vi "Update Icon Textvi.vi"(9 "Icon Color":u32(colorbox)=13631442, 10 "Suubsystem Name":string="Drive", 11 "vi reference":refnum<vi>) -> (3 "VI Refnum out":refnum<vi>)   [LabVIEW 2023]
uses:
  <vilib>/LabVIEW Icon API/lv_icon/Controls/Graphic.ctl
  <vilib>/LabVIEW Icon API/lv_icon/Classes/Layer/Layer.lvclass
  <vilib>/LabVIEW Icon API/lv_icon/Controls/Layer.ctl
  <vilib>/LabVIEW Icon API/lv_icon/Classes/Icon/Icon.lvclass
  <vilib>/LabVIEW Icon API/lv_icon/Classes/Icon Framework/Icon Framework.lvclass
  <vilib>/LabVIEW Icon API/LabVIEW Icon API.lvlib
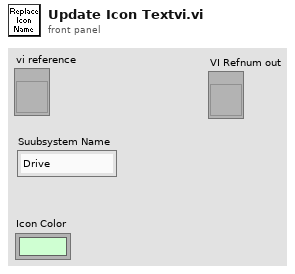
[diagram p1: front panel]
types:
  T1 = typedef "Layer.ctl" = cluster{"LayerIcon":picture, "LayerName":string, "Opacity":u8, "Visibility?":bool}
  T2 = cluster{"left":i16, "top":i16, "right":i16, "bottom":i16}
  T3 = typedef "Graphic.ctl" = cluster{"Rectangle":cluster{"left":i16, "top":i16, "right":i16, "bottom":i16}, "Path":path, "Image":picture, "Filter":string, "FileName":string}
  T4 = typedef "BodyText.ctl" = cluster{"Line 1 text":string, "Line 2 text":string, "Line 3 text":string, "Line 4 text":string, "Line 1 color":u32, "Line 2 color":u32, "Line 3 color":u32, "Line 4 color":u32, "Body Text Spec":cluster{"Font":T5, "Alignment":T6, "Size":u8}, "Center text vertically":bool, "Capitalize Text":bool}
  T5 = typedef "Font.ctl" = string
  T6 = typedef "Alignment.ctl" = u16
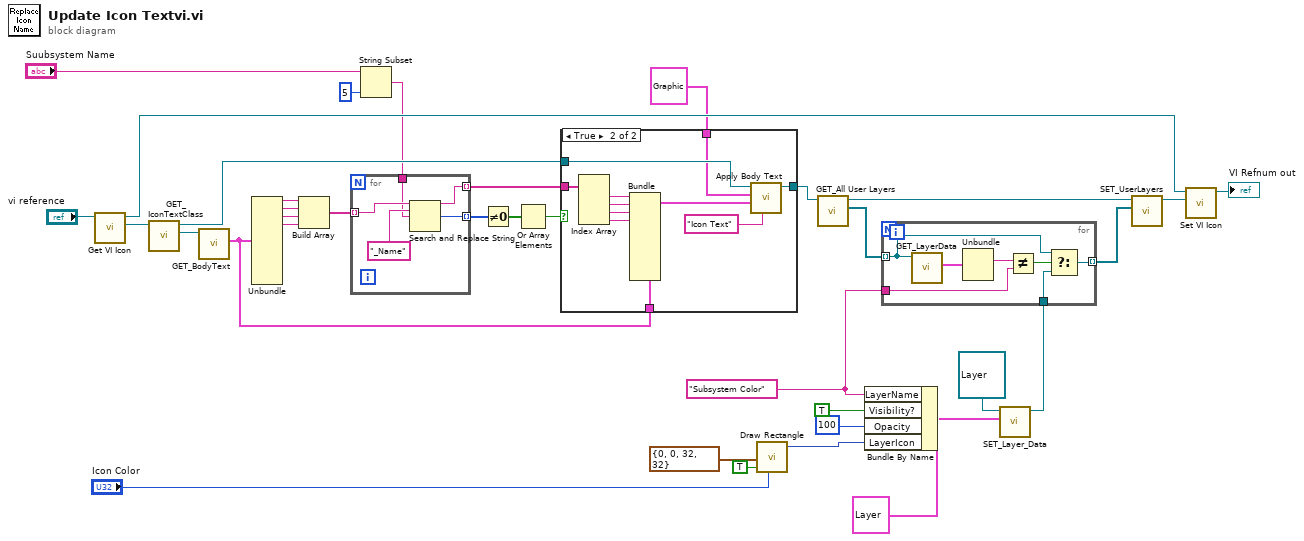
[diagram p0: block diagram]
diagram:
  w3 = "Subsystem Color" ("Layer name")
  n1 = call <vilib>:"Get VI Icon.vi"("VI Refnum in"="vi reference") -> ("Icon"=w36:refnum<class "Icon.lvclass">, "VI Refnum out"=w24:refnum<vi>)  [unwired: 8 in, 1 out]
  n2 = call-dynamic "GET_IconTextClass.vi"("Icon.lvclass in"=w36) -> ("Icon Framework.lvclass"=w35:refnum<class "Icon Framework.lvclass">, "Icon.lvclass out"=w25:refnum<class "Icon.lvclass">)  [unwired: 8 in, 1 out]
  n3 = call-dynamic "GET_BodyText.vi"("Icon Framework.lvclass in"=w35) -> ("Body Text"=w26:T4)  [unwired: 7 in, 3 out]
  n4 = Unbundle(w26) -> ("Line 1 text"=w31:string, "Line 2 text"=w32:string, "Line 3 text"=w33:string, "Line 4 text"=w34:string)  [unwired: 7 out]
  n5 = Build Array(w31, w32, w33, w34) -> (w30:string[])
  n6 = String Subset(string="Suubsystem Name", length (rest)=5 ("length (rest)")) -> (substring=w19:string)  [unwired: 1 in]
  n7 = for {
    tunnel: w30 -> [w40] mode=indexing
    tunnel: w19 -> [w39]
    tunnel: [w38] -> w29 mode=indexing
    tunnel: [w37] -> w27 mode=indexing
    n8 = Search and Replace String(input string=w40, search string="_Name", replace string=w39) -> (result string=w37:string, number of replacements=w38:i32)  [unwired: 5 in, 2 out]
  }
  n9 = Not Equal To 0?(x=w29) -> (x != 0?=w28:bool[])
  n10 = Or Array Elements(Boolean array=w28) -> (logical OR=w5:bool)
  n11 = case shown="True" w5 {
    tunnel: w27 -> [_ w53]
    tunnel: w26 -> [_ w52]
    tunnel: w25 -> [w42 w51]
    tunnel: T3 {"Rectangle"={"left"=0, "top"=0, "right"=0, "bottom"=0}, "Path"=path "", "Image"=bytes[0], "Filter"="", "FileName"=""} ("Path & Icon") -> [_ w50]
    tunnel: [w42 w43] -> w7
    frame False {
    }
    frame True {
      n12 = Index Array(array=w53) -> (element #1=w49:string, element #2=w48:string, element #3=w47:string, element #4=w46:string)  [unwired: 4 in]
      n13 = Bundle(cluster=w52, "Line 1 text"=w49, "Line 2 text"=w48, "Line 3 text"=w47, "Line 4 text"=w46) -> (w45:T4)  [unwired: 7 in]
      n14 = call <vilib>:"Apply Body Text.vi"("Layer name"="Icon Text", "Body test"=w45, "Path & Icon"=w50, "Icon in"=w51) -> ("Icon out"=w43:refnum<class "Icon.lvclass">)  [unwired: 5 in, 2 out]
    }
  }
  n15 = call <vilib>:"Draw Rectangle.vi"("rect"=T2 {"left"=0, "top"=0, "right"=32, "bottom"=32}, "fill?(F)"=TRUE, "color(black)"="Icon Color") -> ("new picture"=w11:picture)  [unwired: 6 in]
  n16 = call-dynamic "GET_All User Layers.vi"("Icon.lvclass in"=w7) -> ("User Layer"=w4:refnum<class "Layer.lvclass">[], "Icon.lvclass out"=w8:refnum<class "Icon.lvclass">)  [unwired: 8 in, 1 out]
  n17 = Bundle By Name(cluster=T1 {"LayerIcon"=bytes[0], "LayerName"="", "Opacity"=0, "Visibility?"=FALSE} ("Data"), "LayerName"=w3, "Visibility?"=TRUE, "Opacity"=u8 100, "LayerIcon"=w11) -> (w9:T1)
  n18 = call-dynamic "SET_Layer_Data.vi"("Data"=w9, "Layer.lvclass in"=refnum<class "Layer.lvclass"> refnum) -> ("Layer.lvclass out"=w2:refnum<class "Layer.lvclass">)  [unwired: 2 in, 7 out]
  n19 = for {
    tunnel: w4 -> [w56] mode=indexing
    tunnel: w3 -> [w59]
    tunnel: w2 -> [w55]
    tunnel: [w54] -> w1 mode=indexing
    n20 = call-dynamic "GET_LayerData.vi"("Layer.lvclass in"=w56) -> ("Data"=w60:T1)  [unwired: 6 in, 4 out]
    n21 = Unbundle(w60) -> ("LayerName"=w58:string)  [unwired: 3 out]
    n22 = Not Equal?(x=w58, y=w59) -> (x != y?=w57:bool)
    n23 = Select(t=w56, s=w57, f=w55) -> (s? t:f=w54:refnum<class "Layer.lvclass">)
  }
  n24 = call-dynamic "SET_UserLayers.vi"("Layers"=w1, "Icon.lvclass in"=w8) -> ("Icon.lvclass out"=w6:refnum<class "Icon.lvclass">)  [unwired: 8 in, 1 out]
  n25 = call <vilib>:"Set VI Icon.vi"("Icon"=w6, "VI Refnum in"=w24) -> ("VI Refnum out"=→"VI Refnum out":refnum<vi>)  [unwired: 8 in, 1 out]
